vi "Read Entries for Day.vi"(7 "Time Entry Store in":refnum<class "Time Entry Store-INI.lvclass">, 8 "error in (no error)":errorcluster, 11 "Date":timestamp) -> (0 "error out":errorcluster, 3 "Time Entries":T1, 5 "Time Entry Store out":refnum<class "Time Entry Store-INI.lvclass">)   [LabVIEW 2024, in "Time Entry Store-INI.lvclass"]
doc: "Returns the time entries whose Start Time falls on the LOCAL calendar day of Date (midnight to midnight in the time zone of the computer), sorted by Start Time. Month files are bucketed by UTC, so two files are read when the local day spans a UTC month boundary.\n\nGenerated by: Claude"
uses:
  Time Entry Store-INI.lvclass
  Time Entry Store-INI.lvclass/Time Entry Store-INI.ctl
  Rows/Time Entry.ctl
  Rows/Time Entry List.ctl
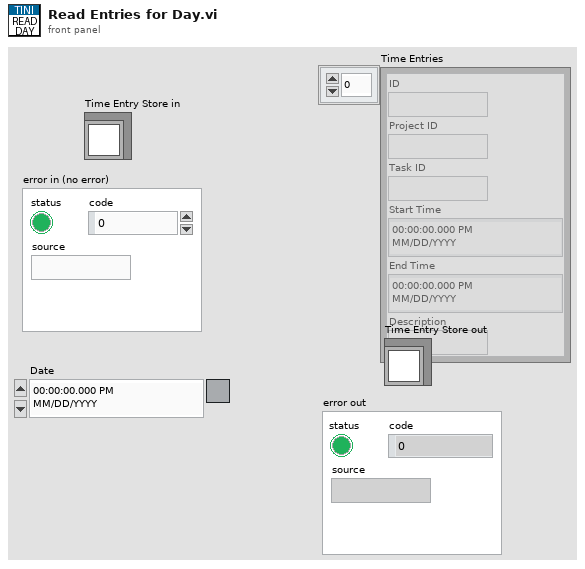
[diagram p1: front panel]
types:
  T1 = typedef "Time Entry List.ctl" = T2[]
  T2 = typedef "Time Entry.ctl" = cluster{"ID":string, "Project ID":string, "Task ID":string, "Start Time":timestamp, "End Time":timestamp, "Description":string}
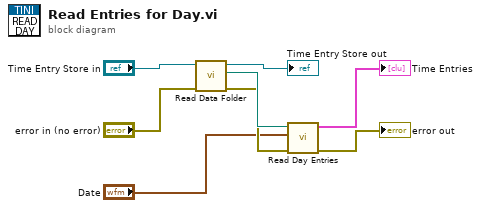
[diagram p0: block diagram]
diagram:
  n1 = call-dynamic "Read Data Folder.vi"("error in (no error)"="error in (no error)", "Time Entry Store-INI in"="Time Entry Store in") -> ("error out"=w4:errorcluster, "Data Folder"=w6:path, "Time Entry Store-INI out"=→"Time Entry Store out":refnum<class "Time Entry Store-INI.lvclass">)  [unwired: 7 in]
  n2 = call "Read Day Entries.vi"("error in (no error)"=w4, "Date"="Date", "Data Folder"=w6) -> ("error out"=→"error out":errorcluster, "Time Entries"=→"Time Entries":T1)  [unwired: 7 in]
